vi "Connect.vi"(4 "Port (22)":u16=22, 6 "Timeout (60000 ms)":i32=60000, 8 "Error In":errorcluster, 10 "Address":string, 11 "Session In":refnum<class "Session.lvclass">) -> (0 "Error Out":errorcluster, 3 "Sesssion Out":refnum<class "Session.lvclass">)   [LabVIEW 2018, in "Toolkit.lvlib" / "Session.lvclass"]
doc: "Connects a sesssion to a remote SSH server. This is typically called immediately after creating the session, and this must be called BEFORE authenticating a user with the remote SSH server."
uses:
  Session.lvclass
  Session.lvclass/Session.ctl
  SSH/SSH.lvclass/SSH.ctl
  Toolkit.lvlib
  SSH/SSH.lvclass
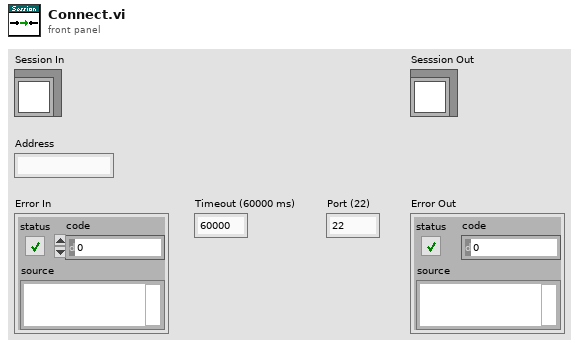
[diagram p1: front panel]
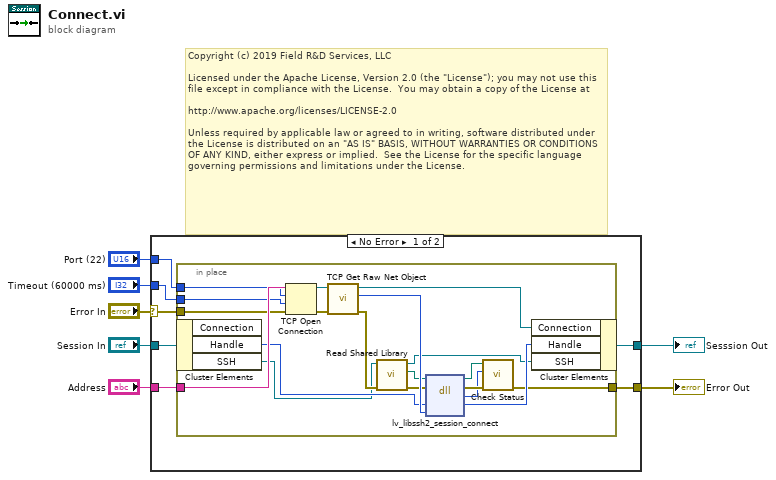
[diagram p0: block diagram]
diagram:
  # "Copyright (c) 2019 Field R&D Services, LLC\n\nLicensed under the Apache License, Version 2.0 (the \"License\"); you may not use this file except in compliance with the License.  You may obtain a copy of the License at\n\nhttp://www.apache.org/licenses/LICENSE-2.0\n\nUnless required by applicable law or agreed to in writing, software distributed under the License is distributed on an \"AS IS\" BASIS, WITHOUT WARRANTIES OR CONDITIONS OF ANY KIND, either express or implied.  See the License for the specific language governing permissions and limitations under the License."
  n1 = case shown="No Error" "Error In" {
    selector: "Error In" -> [w12 w35]
    tunnel: "Address" -> [w14 _]
    tunnel: [w13 w35] -> w5
    tunnel: "Session In" -> [w11 w34]
    tunnel: [w10 w34] -> w3
    tunnel: "Timeout (60000 ms)" -> [w9 _]
    tunnel: "Port (22)" -> [w8 _]
    frame No Error {
      n2 = in-place {
        in-place-border: w14 -> [w33]
        in-place-border: [w22] -> w13
        in-place-border: w12 -> [w32]
        in-place-border: w9 -> [w16]
        in-place-border: w8 -> [w15]
        n3 = in-place-cluster #1(w11) -> ("Handle"=w26:u64, "SSH"=w19:refnum<class "SSH.lvclass">)  [unwired: 1 out]
        n4 = TCP Open Connection(address=w33, remote port or service name=w15, timeout ms (60000)=w16, error in (no error)=w32) -> (connection ID=w30:refnum<k5>, error out=w31:errorcluster)  [unwired: 1 in]
        n5 = call <vilib>:"TCP Get Raw Net Object.vi"("error in (no error)"=w31, "connection ID"=w30) -> ("error out"=w29:errorcluster, "raw net object"=w28:u64, "connection ID out"=w27:refnum<k5>)  [unwired: 7 in]
        n6 = call "Read Shared Library.vi"("Error In"=w29, "SSH In"=w19) -> ("Error Out"=w20:errorcluster, "libssh2lv Shared Library"=w17:path, "SSH Out"=w18:refnum<class "SSH.lvclass">)  [unwired: 7 in]
        n7 = dll-call lib="libssh2lv.*" fn="lv_libssh2_session_connect"(path in=w17, error in=w20, "session"=w26, "socket"=w28) -> (path out=w23:path, error out=w24:errorcluster, "result"=w21:i32, "session"=w25:u64)  [unwired: 2 in]
        n8 = call "Check Status.vi"("Error In"=w24, "Status"=w21, "libssh2lv Shared Library In"=w23) -> ("Error Out"=w22:errorcluster)  [unwired: 7 in, 1 out]
        n9 = in-place-cluster #1("Connection"=w27, "Handle"=w25, "SSH"=w18) -> (w10:refnum<class "Session.lvclass">)
      }
    }
    frame Error {
    }
  }
  "Sesssion Out" <- w3
  "Error Out" <- w5
